vi "Client Received Reply Queue.vi"(11 "创建?":bool) -> (0 "error out":errorcluster caption="错误输出", 3 "queue out":refnum<queue>)   [LabVIEW 2020, in "TCP Communication.lvlib"]
uses:
  TCP Communication.lvlib
  Reply.ctl
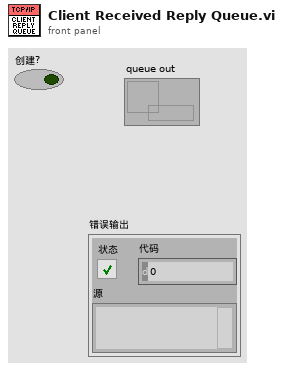
[diagram p1: front panel]
types:
  T1 = typedef "TCP Communication.lvlib/Reply.ctl" = cluster{"ID":i32, "CMD":string, "Data":variant}
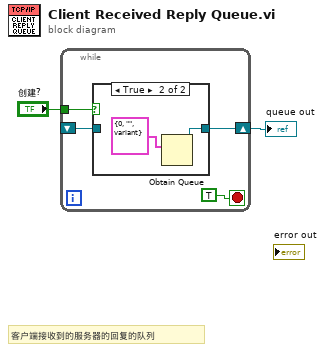
[diagram p0: block diagram]
diagram:
  # "客户端接收到的服务器的回复的队列"
  n1 = while {
    tunnel: "创建?" -> [w5]
    shift-right: [w3] -> w1
    shift-left: _ -> [w4]
    stop <- TRUE stop-if-true
    n2 = case shown="True" w5 {
      tunnel: [w7 w8] -> w3
      tunnel: w4 -> [w7 _]
      frame False {
      }
      frame True {
        n3 = Obtain Queue(element data type=T1 {"ID"=0, "CMD"="", "Data"=variant} ("回复")) -> (queue out=w8:refnum<queue>)  [unwired: 4 in, 2 out]
      }
    }
  }
  "queue out" <- w1
